vi "myFreqGroup.vi"(6 "基波频率":u32=50, 7 "最大同时扫频数":u32=7, 8 "响应端口额外频率位移":i8(ring) items=["-2次基波"=-2, "-1次基波"=-1, "无位移"=0, "+1次基波"=1, "+2次基波"=2, "对称-2次基波"=98, "对称-1次基波"=99, "对称"=100, "对称+1次基波"=101, "对称+2次基波"=102], 9 "响应(2号)端口类型":u8(ring) items=["单相", "三相αβ系", "三相同步系", "三相正负序"], 10 "注入(1号)端口类型":u8(ring) items=["单相", "三相αβ系", "三相同步系", "三相正负序"], 11 "freqs_measu_coups":i32[][](array[numeric])) -> (1 "index group":i32[][](array[numeric]), 2 "freqs groups 3D":i32[][][](array[numeric]))   [LabVIEW 2024]
doc: "根据 1D freqs 生成解耦的频率组 3D freqs_group，\n第0维：freqs group，它的每行是需要同时注入的频点，空位用0补齐表示无效。\n1: measu group\n2: coups group\n3: index group，是从 freqs_group 到 freqs 寻址时的对应索引 2D 数组。\n支持负频率。"
uses:
  44807d3e-8a65-4df4-be66-e046820cc363.vi
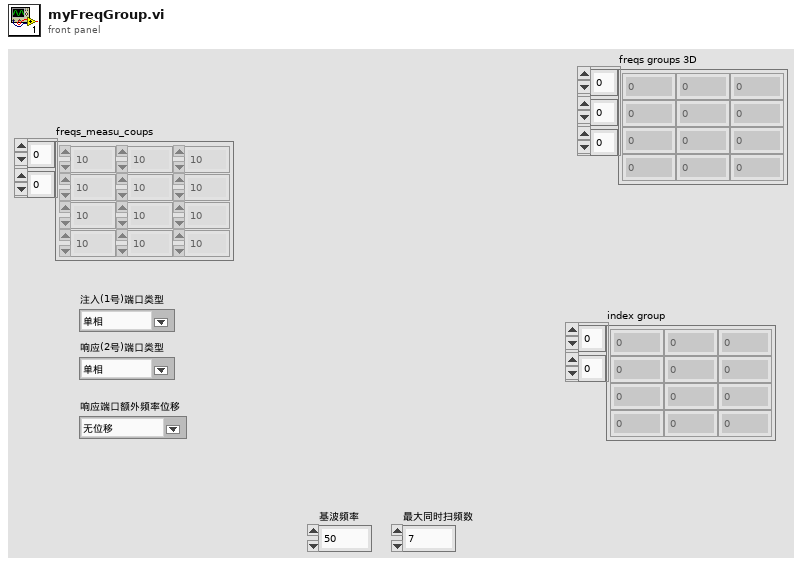
[diagram p1: front panel]
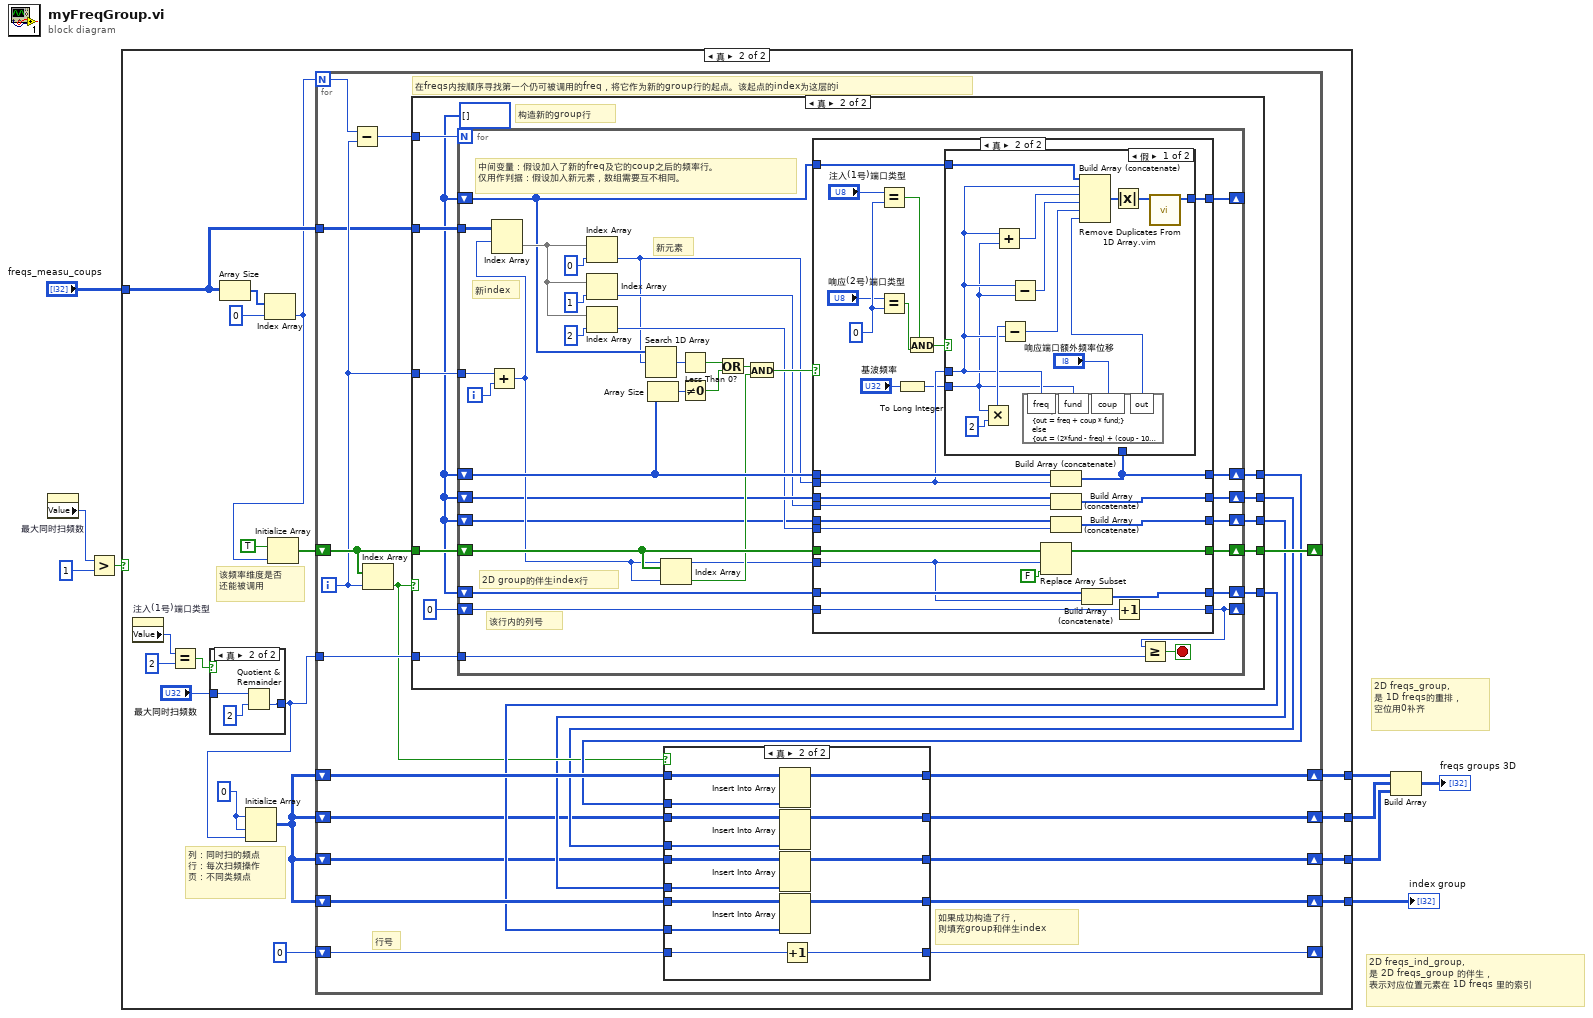
[diagram p0: block diagram]
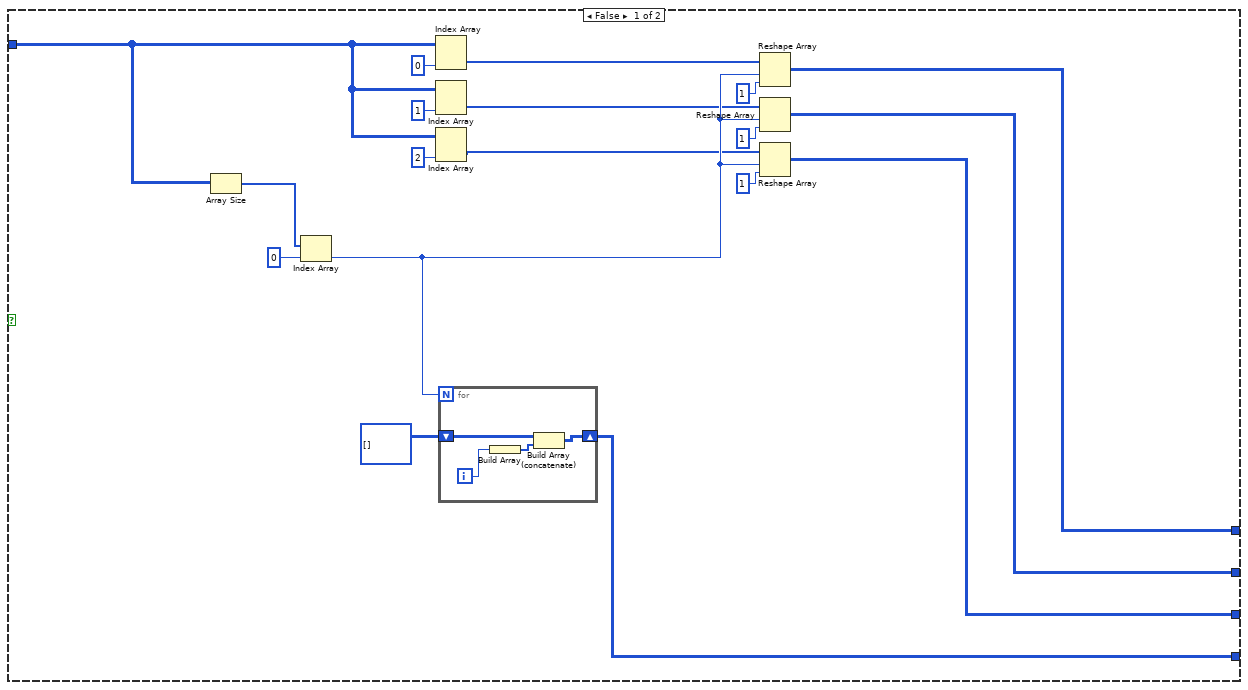
[diagram p2: hidden frame]
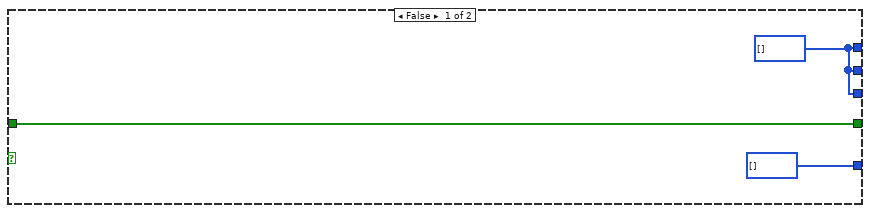
[diagram p5: hidden frame]
diagram:
  # "2D freqs_ind_group,\n是 2D freqs_group 的伴生，\n表示对应位置元素在 1D freqs 里的索引"
  # "2D freqs_group,\n是 1D freqs的重排，\n空位用0补齐"
  n1 = property on="最大同时扫频数" class="DigNum (严格)"() -> ("Value"=w9:u32)  [unwired: 2 in, 2 out]
  n2 = Greater?(x=w9, y=u32 1) -> (0:w7:bool)
  n3 = case shown="真" w7 {
    tunnel: [w26 w47] -> w5
    tunnel: [w24 w46] -> w1
    tunnel: "freqs_measu_coups" -> [w17 w40]
    tunnel: [w10 w34] -> w3
    tunnel: [w11 w33] -> w4
    frame False {
      n4 = Array Size(array=w17) -> (size(s)=w21:i32[])
      n5 = Index Array(array=w21, index=0 ("索引")) -> (element=w14:i32)
      n6 = Index Array(array=w17, index (col)=0 ("索引")) -> (element=w22:i32[])  [unwired: 1 in]
      n7 = Index Array(array=w17, index (col)=1 ("索引")) -> (element=w13:i32[])  [unwired: 1 in]
      n8 = Index Array(array=w17, index (col)=2 ("索引")) -> (element=w12:i32[])  [unwired: 1 in]
      n9 = for {
        N: w14 -> [_]
        shift-right: [w30] -> w24
        shift-left: i32[][] [] -> [w31]
        i -> [w29]
        n10 = Build Array(w29) -> (w28:i32[])
        n11 = Build Array (concatenate)(w31, w28) -> (w30:i32[][])
      }
      n12 = Reshape Array(w22, w14, 1) -> (w26:i32[][])
      n13 = Reshape Array(w13, w14, 1) -> (w11:i32[][])
      n14 = Reshape Array(w12, w14, 1) -> (w10:i32[][])
    }
    frame True {
      w45 = 0
      # "列：同时扫的频点\n行：每次扫频操作\n页：不同类频点"
      # "该频率维度是否\n还能被调用"
      n15 = property on="注入(1号)端口类型" class="Ring (严格)"() -> ("Value"=w41:u8)  [unwired: 2 in, 2 out]
      n16 = Equal?(x=w41, y=u8 2) -> (x = y?=w42:bool)
      n17 = case shown="真" w42 {
        tunnel: "最大同时扫频数" -> [w50 w52]
        tunnel: [w50 w51] -> w32
        frame False {
        }
        frame True {
          n18 = Quotient & Remainder(x=w52, y=2) -> (floor(x/y)=w51:u32)  [unwired: 1 out]
        }
      }
      n19 = Array Size(array=w40) -> (size(s)=w39:i32[])
      n20 = Initialize Array(w45, w45, w32) -> (w35:i32[][])
      n21 = Index Array(array=w39, index=0 ("索引")) -> (element=w37:i32)
      n22 = Initialize Array(TRUE, w37) -> (w48:bool[])
      n23 = for {
        N: w37 -> [w70]
        shift-right: [w72] -> w47
        shift-left: w35 -> [w73]
        shift-right: [w74] -> _
        shift-left: w48 -> [w69]
        shift-right: [w67] -> w46
        shift-left: w35 -> [w66]
        tunnel: w32 -> [w64]
        tunnel: w40 -> [w62]
        shift-right: [w60] -> _
        shift-left: 0 -> [w61]
        shift-right: [w55] -> w33
        shift-left: w35 -> [w56]
        shift-right: [w54] -> w34
        shift-left: w35 -> [w57]
        i -> [w68]
        # "如果成功构造了行，\n则填充group和伴生index"
        # "行号"
        # "在freqs内按顺序寻找第一个仍可被调用的freq，将它作为新的group行的起点。该起点的index为这层的i"
        n24 = Subtract(x=w70, y=w68) -> (x-y=w75:i32)
        n25 = Index Array(array=w69, index=w68) -> (element=w63:bool)
        n26 = case shown="真" w63 {
          tunnel: w69 -> [w97 w108]
          tunnel: w75 -> [_ w103]
          tunnel: w68 -> [_ w109]
          tunnel: [w97 w107] -> w74
          tunnel: [w95 w106] -> w71
          tunnel: [i32[] [] w104] -> w65
          tunnel: w64 -> [_ w102]
          tunnel: w62 -> [_ w101]
          tunnel: [w95 w99] -> w59
          tunnel: [w95 w98] -> w58
          frame False {
            w95 = i32[] []
          }
          frame True {
            w100 = i32[] []
            # "构造新的group行"
            n27 = for {
              N: w103 -> [_]
              shift-right: [w137] -> w106
              shift-left: w100 -> [w139]
              tunnel: w109 -> [w143]
              shift-right: [w141] -> w107
              shift-left: w108 -> [w136]
              shift-right: [w138] -> _
              shift-left: w100 -> [w111]
              shift-right: [w132] -> _
              shift-left: 0 -> [w133]
              shift-right: [w134] -> w104
              shift-left: w100 -> [w135]
              tunnel: w102 -> [w130]
              tunnel: w101 -> [w123]
              shift-right: [w119] -> w99
              shift-left: w100 -> [w120]
              shift-right: [w112] -> w98
              shift-left: w100 -> [w113]
              i -> [w142]
              stop <- w131 stop-if-true
              # "新index"
              # "该行内的列号"
              # "2D group的伴生index行"
              # "中间变量：假设加入了新的freq及它的coup之后的频率行。\n仅用作判据：假设加入新元素，数组需要互不相同。"
              # "新元素"
              n28 = Add(x=w143, y=w142) -> (x+y=w122:i32)
              n29 = Index Array(array=w123, index (row)=w122) -> (element=w116:i32[])  [unwired: 1 in]
              n30 = Index Array(array=w116, index=0 ("索引")) -> (element=w110:i32)
              n31 = Index Array(array=w116, index=1 ("索引")) -> (element=w114:i32)
              n32 = Index Array(array=w116, index=2 ("索引")) -> (element=w115:i32)
              n33 = Search 1D Array(1D array=w111, element=w110) -> (index of element=w129:i32)  [unwired: 1 in]
              n34 = Array Size(array=w139) -> (size(s)=w140:i32)
              n35 = Index Array(array=w136, index=w122) -> (element=w128:bool)
              n36 = Less Than 0?(x=w129) -> (x < 0?=w125:bool)
              n37 = Not Equal To 0?(x=w140) -> (x != 0?=w124:bool)
              n38 = Or(x=w125, y=w124) -> (x .or. y?=w126:bool)
              n39 = And(x=w126, y=w128) -> (x .and. y?=w127:bool)
              n40 = case shown="真" w127 {
                tunnel: w139 -> [w150 w174]
                tunnel: w110 -> [_ w159]
                tunnel: [w150 w162] -> w137
                tunnel: w136 -> [w149 w177]
                tunnel: w122 -> [_ w169]
                tunnel: [w149 w175] -> w141
                tunnel: w111 -> [w148 w160]
                tunnel: [w148 w161] -> w138
                tunnel: w133 -> [w147 w172]
                tunnel: [w147 w173] -> w132
                tunnel: w135 -> [w146 w171]
                tunnel: [w146 w170] -> w134
                tunnel: w115 -> [_ w154]
                tunnel: w120 -> [w145 w156]
                tunnel: [w145 w155] -> w119
                tunnel: w114 -> [_ w152]
                tunnel: w113 -> [w144 w153]
                tunnel: [w144 w151] -> w112
                frame False {
                }
                frame True {
                  w168 = u8 0
                  n41 = Equal?(x="注入(1号)端口类型", y=w168) -> (x = y?=w165:bool)
                  n42 = Equal?(x="响应(2号)端口类型", y=w168) -> (x = y?=w164:bool)
                  n43 = To Long Integer(number="基波频率") -> (32bit integer=w157:i32)
                  n44 = And(x=w165, y=w164) -> (x .and. y?=w163:bool)
                  n45 = Replace Array Subset(array=w177, new element=FALSE, index=w169) -> (w175:bool[])
                  n46 = Build Array (concatenate)(w174, w159) -> (w162:i32[])
                  n47 = case shown="假" w163 {
                    tunnel: w162 -> [_ w191]
                    tunnel: [w179 w191] -> w161
                    tunnel: w160 -> [w183 _]
                    tunnel: w159 -> [w182 _]
                    tunnel: w157 -> [w178 _]
                    frame False {
                      n48 = Multiply(x=w178, y=2) -> (x*y=w189:i32)
                      n49 = Add(x=w182, y=w178) -> (x+y=w184:i32)
                      n50 = Subtract(x=w189, y=w182) -> (x-y=w186:i32)
                      n51 = Subtract(x=w182, y=w178) -> (x-y=w185:i32)
                      n52 = formula code="int out;\nif(coup < 50)\n{out = freq + coup * fund;}\nelse\n{out = (2*fund - freq) + (coup - 100) * fund;}"("coup"="响应端口额外频率位移", "freq"=w182, "fund"=w178) -> ("out"=w187:i32)
                      n53 = Build Array (concatenate)(w183, w182, w184, w185, w186, w187) -> (w181:i32[])
                      n54 = Absolute Value(x=w181) -> (abs(x)=w180:i32[])
                      n55 = call "Remove Duplicates From 1D Array.vim"("array"=w180) -> ("array with duplicates removed"=w179:i32[])  [unwired: 10 in]
                    }
                    frame True {
                    }
                  }
                  n56 = Build Array (concatenate)(w156, w152) -> (w155:i32[])
                  n57 = Build Array (concatenate)(w153, w154) -> (w151:i32[])
                  n58 = Build Array (concatenate)(w171, w169) -> (w170:i32[])
                  n59 = Increment(x=w172) -> (x+1=w173:i32)
                }
              }
              n60 = Greater Or Equal?(x=w132, y=w130) -> (x >= y?=w131:bool)
            }
          }
        }
        n61 = case shown="真" w63 {
          tunnel: w73 -> [w80 w90]
          tunnel: w71 -> [_ w93]
          tunnel: [w80 w94] -> w72
          tunnel: [w79 w92] -> w67
          tunnel: w66 -> [w79 w89]
          tunnel: w65 -> [_ w91]
          tunnel: w61 -> [w78 w82]
          tunnel: [w78 w81] -> w60
          tunnel: w59 -> [_ w88]
          tunnel: w58 -> [_ w87]
          tunnel: w57 -> [w77 w86]
          tunnel: w56 -> [w76 w85]
          tunnel: [w76 w84] -> w55
          tunnel: [w77 w83] -> w54
          frame False {
          }
          frame True {
            n62 = Insert Into Array(array=w90, new element=w93) -> (w94:i32[][])  [unwired: 2 in]
            n63 = Insert Into Array(array=w85, new element=w88) -> (w84:i32[][])  [unwired: 2 in]
            n64 = Insert Into Array(array=w86, new element=w87) -> (w83:i32[][])  [unwired: 2 in]
            n65 = Insert Into Array(array=w89, new element=w91) -> (w92:i32[][])  [unwired: 2 in]
            n66 = Increment(x=w82) -> (x+1=w81:i32)
          }
        }
      }
    }
  }
  "index group" <- w1
  n67 = Build Array(w5, w4, w3) -> (→"freqs groups 3D":i32[][][])
